vi "Read Address.vi"(11 "Notifier Transport in":refnum<class "Notifier Transport.lvclass">) -> (2 "Address":refnum<data-value>)   [LabVIEW 2020, in "jettl.lvlib" / "Notifier Transport.lvlib" / "Notifier Transport.lvclass"]
uses:
  Notifier Transport.lvclass
  Msg/Msg.lvclass
  Notifier Transport.lvclass/Notifier Transport.ctl
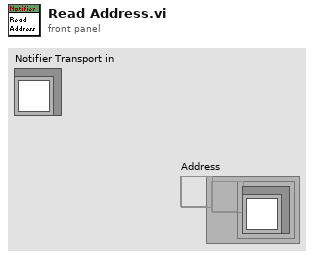
[diagram p1: front panel]
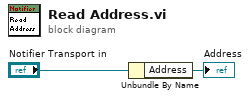
[diagram p0: block diagram]
diagram:
  n1 = Unbundle By Name("Notifier Transport in") -> ("Address"=→"Address":refnum<data-value>)
